vi "Reject Non Object Message.vi"(8 "error in":errorcluster, 10 "response":string, 11 "request":string) -> (0 "error out":errorcluster, 3 "response out":string)   [LabVIEW 2020, in "MCP Server.lvlib"]
doc: "A JSON-RPC message has to be a JSON object. If the received text is valid JSON but not an object (an array, a string, a number, true, false or null), the answer is JSON-RPC error -32600 (Invalid Request) with id null.\n\nEvery other response is passed through: an object is handled by the caller, and text that is not valid JSON keeps its -32700 (Parse error) answer. An array counts as valid only if it ends with its closing bracket."
uses:
  MCP Server.lvlib
  <vilib>/JDP Science/JSONtext/JSONtext.lvlib
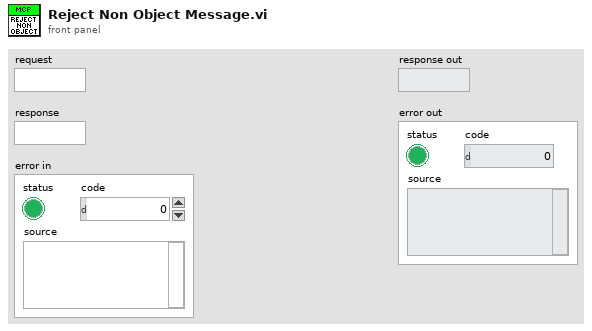
[diagram p1: front panel]
types:
  T1 = typedef "JSONtext.lvlib/JSON Value Type.ctl" = enum16{"Not a JSON Value", "JSON Object", "JSON Array", "String", "Number", "true", "false", "null"}
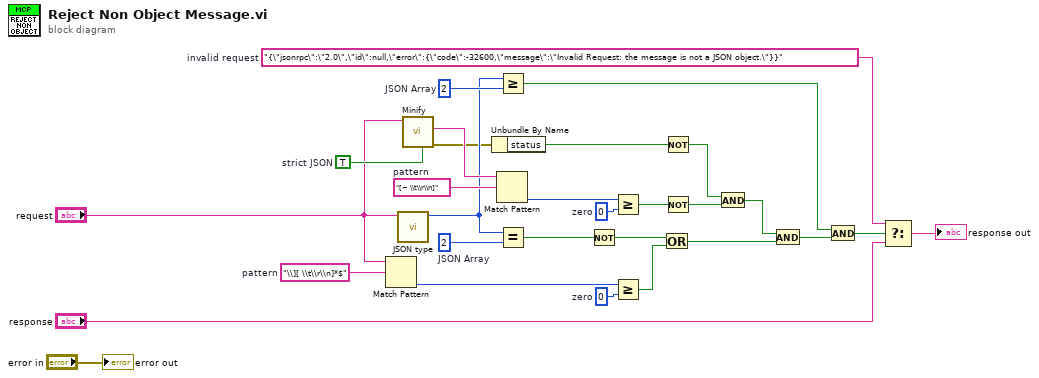
[diagram p0: block diagram]
diagram:
  w5 = "{\"jsonrpc\":\"2.0\",\"id\":null,\"error\":{\"code\":-32600,\"message\":\"Invalid Request: the message is not a JSON object.\"}}"  # invalid request
  w16 = 0  # zero
  w18 = "\\][ \\t\\r\\n]*$"  # pattern
  w21 = u16 2  # JSON Array
  w24 = 0  # zero
  w26 = "[~ \\t\\r\\n]"  # pattern
  w28 = TRUE  # strict JSON
  w29 = u16 2  # JSON Array
  n1 = Match Pattern(string="request", regular expression=w18) -> (offset past match=w17:i32)  [unwired: 1 in, 3 out]
  n2 = call <vilib>:"JSON type.vi"("JSON"="request") -> ("JSON Value Type"=w22:T1)  [unwired: 9 in, 1 out]
  n3 = call <vilib>:"Minify.vi"("Disable LabVIEW Extensions"=w28, "JSON"="request") -> ("error out"=w13:errorcluster, "Rest of Input String"=w27:string)  [unwired: 7 in, 1 out]
  n4 = Unbundle By Name(w13) -> ("status"=w12:bool)
  n5 = Match Pattern(string=w27, regular expression=w26) -> (offset past match=w25:i32)  [unwired: 1 in, 3 out]
  n6 = Greater Or Equal?(x=w22, y=w29) -> (x >= y?=w7:bool)
  n7 = Equal?(x=w22, y=w21) -> (x = y?=w20:bool)
  n8 = Not(x=w20) -> (.not. x?=w15:bool)
  n9 = Greater Or Equal?(x=w25, y=w24) -> (x >= y?=w23:bool)
  n10 = Greater Or Equal?(x=w17, y=w16) -> (x >= y?=w14:bool)
  n11 = Or(x=w15, y=w14) -> (x .or. y?=w8:bool)
  n12 = Not(x=w12) -> (.not. x?=w11:bool)
  n13 = Not(x=w23) -> (.not. x?=w10:bool)
  n14 = And(x=w11, y=w10) -> (x .and. y?=w9:bool)
  n15 = And(x=w9, y=w8) -> (x .and. y?=w6:bool)
  n16 = And(x=w7, y=w6) -> (x .and. y?=w4:bool)
  n17 = Select(t=w5, s=w4, f="response") -> (s? t:f=→"response out":string)
  "error out" <- "error in"
